vi "VM3 - Read Variables (ANY).vi"(6 "atomic (F)":bool, 7 "VC Handle":T4, 8 "error in":errorcluster, 11 "name_specs":string[](array[string])) -> (0 "error out":errorcluster, 1 "stats":T1[](array[typedef]), 2 "values out":T2(array[cluster]), 3 "dup name_specs":string[](array[string]), 4 "errCodes":T3[](array[typedef]) items=["No error", "Invalid variable type", "Variable not found", "Variable already exists", "Invalid context handle", "Input error", "Invalid data format", "No history attached", "History already attached", "Invalid history parameters", "Wrong variable name", "Wrong alias name", "Non-unique alias", "Alias not found", "No alias associated", "Alias already associated", "Wrong context name", "Non-unique context name", "Context name not found", "Invalid parameter", "Generic error", "Memory Full", "Unrecognized LV error", "Unknown error code"])   [LabVIEW 2021]
doc: "This VI reads multiple variables of arbitrary data types; both predefined and user-defined data types are supported. Refer to the VI Help for more details.\n\n<b>VC Handle</b> specifies the handle of the variable context. To operate on a global variable, pass -1 to this input. \n<b>name_specs</b> defines the name specifiers of the target variables; usually, a name specifier is merely a variable name (see the VI Help for more options).\n\n<b>atomic (F)</b>, if TRUE, guarantees that all variables are read in an atomic transaction. This prevents other VIs or threads from modifying the variables during execution.\n\n<b>values out</b> returns the variable values. An element of this array is a cluster with three members:\n (1) <b>datatype</b> defines a variable data type code.\n (2) <b>DBL</b> contains a variable value of the <b>DBL Number</b> type.\n (3) <b>STR</b> contains a variable value for all other data types; the value is represented in the Flattened-To-String format with the exception of the String data type.\n\n<b>stats</b> returns additional information about the variable values, such as their Writer ID, update time, and update counter.\n\n<b>errCodes</b> returns VarMan error codes individually for each variable. If any element in this array is non-zero, the <b>error out</b> cluster returns the corresponding error description.\n\n::: CalcExpress Toolkit :::\nCopyright (c) 2000-2026 Konstantin Shifershteyn. All rights reserved."
uses:
  cetypes.llb/VarMan Variable Context Handle.ctl
  cetypes.llb/VarMan Error Code.ctl
  cetypes.llb/VarMan Variable Data Statistics.ctl
  cersrc/celveng32.dll
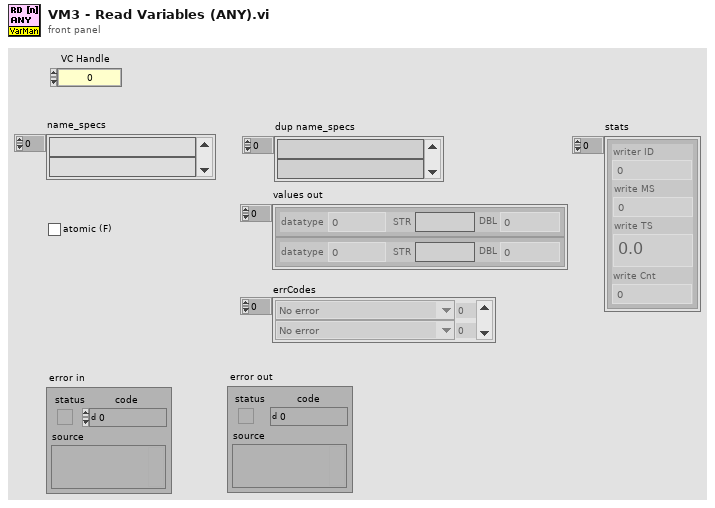
[diagram p1: front panel]
types:
  T1 = typedef "VarMan Variable Data Statistics.ctl" = cluster{"writer ID":u32, "write MS":u32, "write TS":dbl, "write Cnt":u32}
  T2 = cluster{"datatype":u32, "STR":string, "DBL":dbl}[]
  T3 = typedef "VarMan Error Code.ctl" = u16
  T4 = typedef "VarMan Variable Context Handle.ctl" = i32
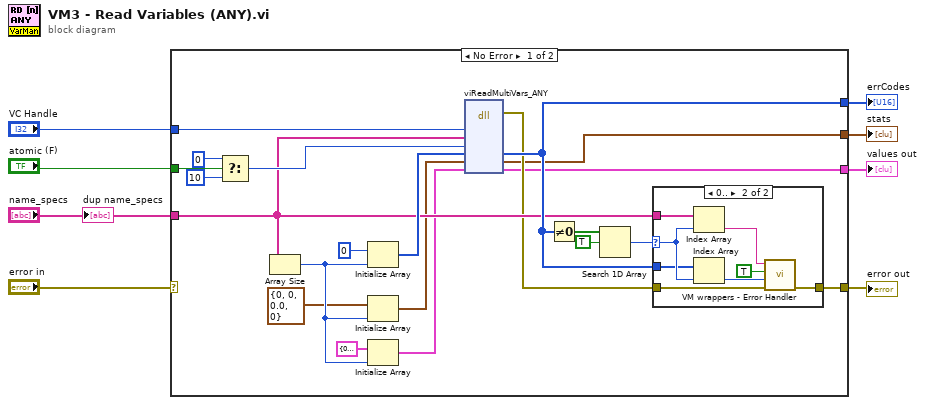
[diagram p0: block diagram]
diagram:
  n1 = case shown="No Error" "error in" {
    selector: "error in" -> [_ w39]
    tunnel: [w19 w39] -> w7
    tunnel: "VC Handle" -> [w29 _]
    tunnel: "name_specs" -> [w21 _]
    tunnel: "atomic (F)" -> [w27 _]
    tunnel: [w22 _] -> w4
    tunnel: [w10 _] -> w3
    tunnel: [w11 _] -> w1
    frame No Error {
      n2 = Select(t=0, s=w27, f=10) -> (s? t:f=w25:i32)
      n3 = Array Size(array=w21) -> (size(s)=w15:i32)
      n4 = Initialize Array(u16 0 ("element"), w15) -> (w23:u16[])
      n5 = Initialize Array(T1 {"writer ID"=0, "write MS"=0, "write TS"=0.0, "write Cnt"=0} ("stats"), w15) -> (w13:T1[])
      n6 = Initialize Array(cluster{"datatype":u32, "STR":string, "DBL":dbl} {"datatype"=0, "STR"="", "DBL"=0.0} ("Cluster"), w15) -> (w12:T2)
      n7 = dll-call lib="C:/LV Projects/CalcExpress 40 LV2021/vi.lib/addons/CalcExpress/cersrc/celveng*.dll" fn="viReadMultiVars_ANY"("vch"=w29, "names"=w21, "lock_cycle"=w25, "errCodes"=w23, "wrStats"=w13, "values"=w12) -> (error out=w20:errorcluster, "errCodes"=w22:u16[], "wrStats"=w11:T1[], "values"=w10:T2)  [unwired: 7 in, 1 out]
      n8 = Not Equal To 0?(x=w22) -> (x != 0?=w18:bool[])
      n9 = Search 1D Array(1D array=w18, element=TRUE) -> (index of element=w16:i32)  [unwired: 1 in]
      n10 = case shown="0.." w16 {
        selector: w16 -> [_ w38]
        tunnel: w22 -> [_ w37]
        tunnel: w21 -> [_ w34]
        tunnel: w20 -> [w30 w32]
        tunnel: [w30 w31] -> w19
        frame ..-1 {
        }
        frame 0.. {
          n11 = Index Array(array=w34, index=w38) -> (element=w33:string)
          n12 = Index Array(array=w37, index=w38) -> (element=w36:u16)
          n13 = call "VM wrappers - Error Handler.vi"("error before"=w32, "VarMan error"=w36, "show name spec (F)"=TRUE, "name spec"=w33) -> ("error out"=w31:errorcluster)  [unwired: 6 in, 1 out]
        }
      }
    }
    frame Error {
    }
  }
  "error out" <- w7
  "errCodes" <- w4
  "values out" <- w3
  "stats" <- w1
  "dup name_specs" <- "name_specs"
